vi "Create Sequence View.vi"(8 "error in (no error)":errorcluster, 10 "Subpanel":refnum<vi>, 11 "TSnax UI Manager in":refnum<class "TSnax UI Manager.lvclass">) -> (0 "error out":errorcluster, 2 "Sequence View":refnum<class "SequenceViewPanel.lvclass">, 3 "TSnax UI Manager out":refnum<class "TSnax UI Manager.lvclass">)   [LabVIEW 2020, in "TSnax UI.lvlib" / "TSnax UI Manager.lvclass"]
uses:
  TSnax UI Manager.lvclass
  SequenceViewPanel/SequenceViewPanel.lvclass
  C:/Program Files (x86)/National Instruments/LabVIEW 2020/vi.lib/IlluminatedG/IG OOPanel/OOPanel/Panel/Panel.lvclass
  TSnax UI Manager.lvclass/TSnax UI Manager.ctl
  <vilib>/IlluminatedG/IG OOPanel/OOPanel/Manager/Manager.lvclass
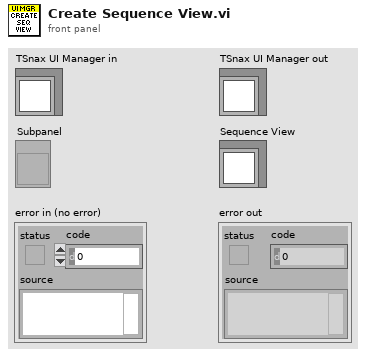
[diagram p1: front panel]
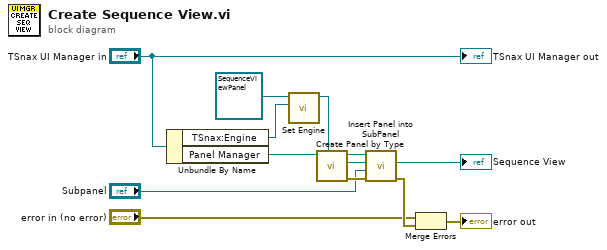
[diagram p0: block diagram]
diagram:
  n1 = Unbundle By Name("TSnax UI Manager in") -> ("TSnax:Engine"=w1:refnum<class "Engine.lvclass">, "Panel Manager"=w13:refnum<class "Manager.lvclass">)
  n2 = call "Set Engine.vi"("TSnax:Engine"=w1, "SequenceViewPanel in"=refnum<class "SequenceViewPanel.lvclass"> refnum ("Sequence View")) -> ("SequenceViewPanel out"=w2:refnum<class "SequenceViewPanel.lvclass">)  [unwired: 8 in, 1 out]
  n3 = call <vilib>:"Create Panel by Type.vi"("Panel Type"=w2, "Manager in"=w13) -> ("error out"=w10:errorcluster, "Panel"=w11:refnum<class "SequenceViewPanel.lvclass">, "Manager out"=w12:refnum<class "Manager.lvclass">)  [unwired: 7 in]
  n4 = call <vilib>:"Insert Panel into SubPanel.vi"("error in (no error)"=w10, "SubPanel"="Subpanel", "Panel In"=w11, "Manager in"=w12) -> ("error out"=w9:errorcluster, "Panel"=→"Sequence View":refnum<class "SequenceViewPanel.lvclass">)  [unwired: 5 in, 1 out]
  n5 = Merge Errors("error in (no error)", w9) -> (→"error out":errorcluster)
  "TSnax UI Manager out" <- "TSnax UI Manager in"
